vi "Locate Array Index.vi"(9 "Top Height":i32, 10 "Row Height":i32, 11 "Array in":refnum<vi>) -> (3 "Index":i32)   [LabVIEW 2020, in "Data Viewer.lvlib"]
uses:
  Data Viewer.lvlib
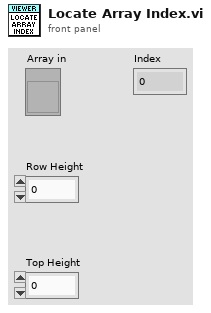
[diagram p1: front panel]
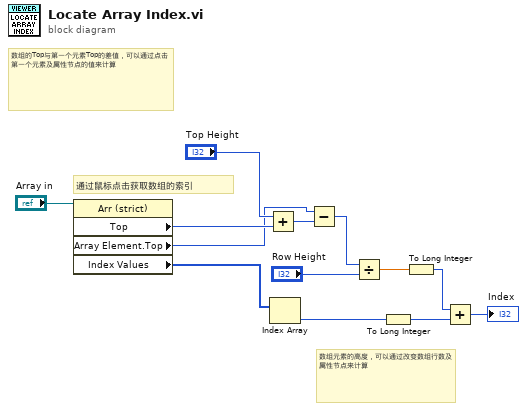
[diagram p0: block diagram]
diagram:
  # "数组元素的高度，可以通过改变数组行数及属性节点来计算"
  # "数组的Top与第一个元素Top的差值，可以通过点击第一个元素及属性节点的值来计算"
  # "通过鼠标点击获取数组的索引"
  n1 = property class="Arr (strict)"(reference="Array in") -> ("Top"=w11:i32, "Array Element.Top"=w4:i32, "Index Values"=w3:u32[])  [unwired: 1 in, 2 out]
  n2 = Add(x="Top Height", y=w11) -> (x+y=w10:i32)
  n3 = Index Array(array=w3) -> (element=w9:u32)  [unwired: 1 in]
  n4 = Subtract(x=w4, y=w10) -> (x-y=w5:i32)
  n5 = Divide(x=w5, y="Row Height") -> (x/y=w7:dbl)
  n6 = To Long Integer(number=w9) -> (32bit integer=w1:i32)
  n7 = To Long Integer(number=w7) -> (32bit integer=w8:i32)
  n8 = Add(x=w8, y=w1) -> (x+y=→"Index":i32)
